vi "GOOP_VI_Item_OnPopupMenu.vi"(11 "Object":u64) -> ()   [LabVIEW 2020]
uses:
  <resource>/Framework/Providers/API/mxLvMenuItem.ctl
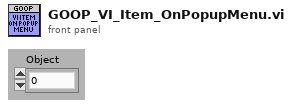
[diagram p1: front panel]
types:
  T1 = typedef "mxLvMenuItem.ctl" = cluster{"Menu Name":string, "Description":string, "Icon File Name":path, "Menu Tag":string, "Enabled":bool, "Checked":bool, "Separator":bool, "Batchable":bool, "Weight":i32, "Batch Mode (Ignored if Not Batchable)":enum32{"Show If All Items Support Command", "Show If Any Items Support Command"}, "Menu Location":enum32{"<None>", "Project", "Project / Build Specifications", "Tools", "Tools / Source Control", "Tools / Real-Time Module", "Help"}, "Exclude From Getting Started Window Menu":bool}
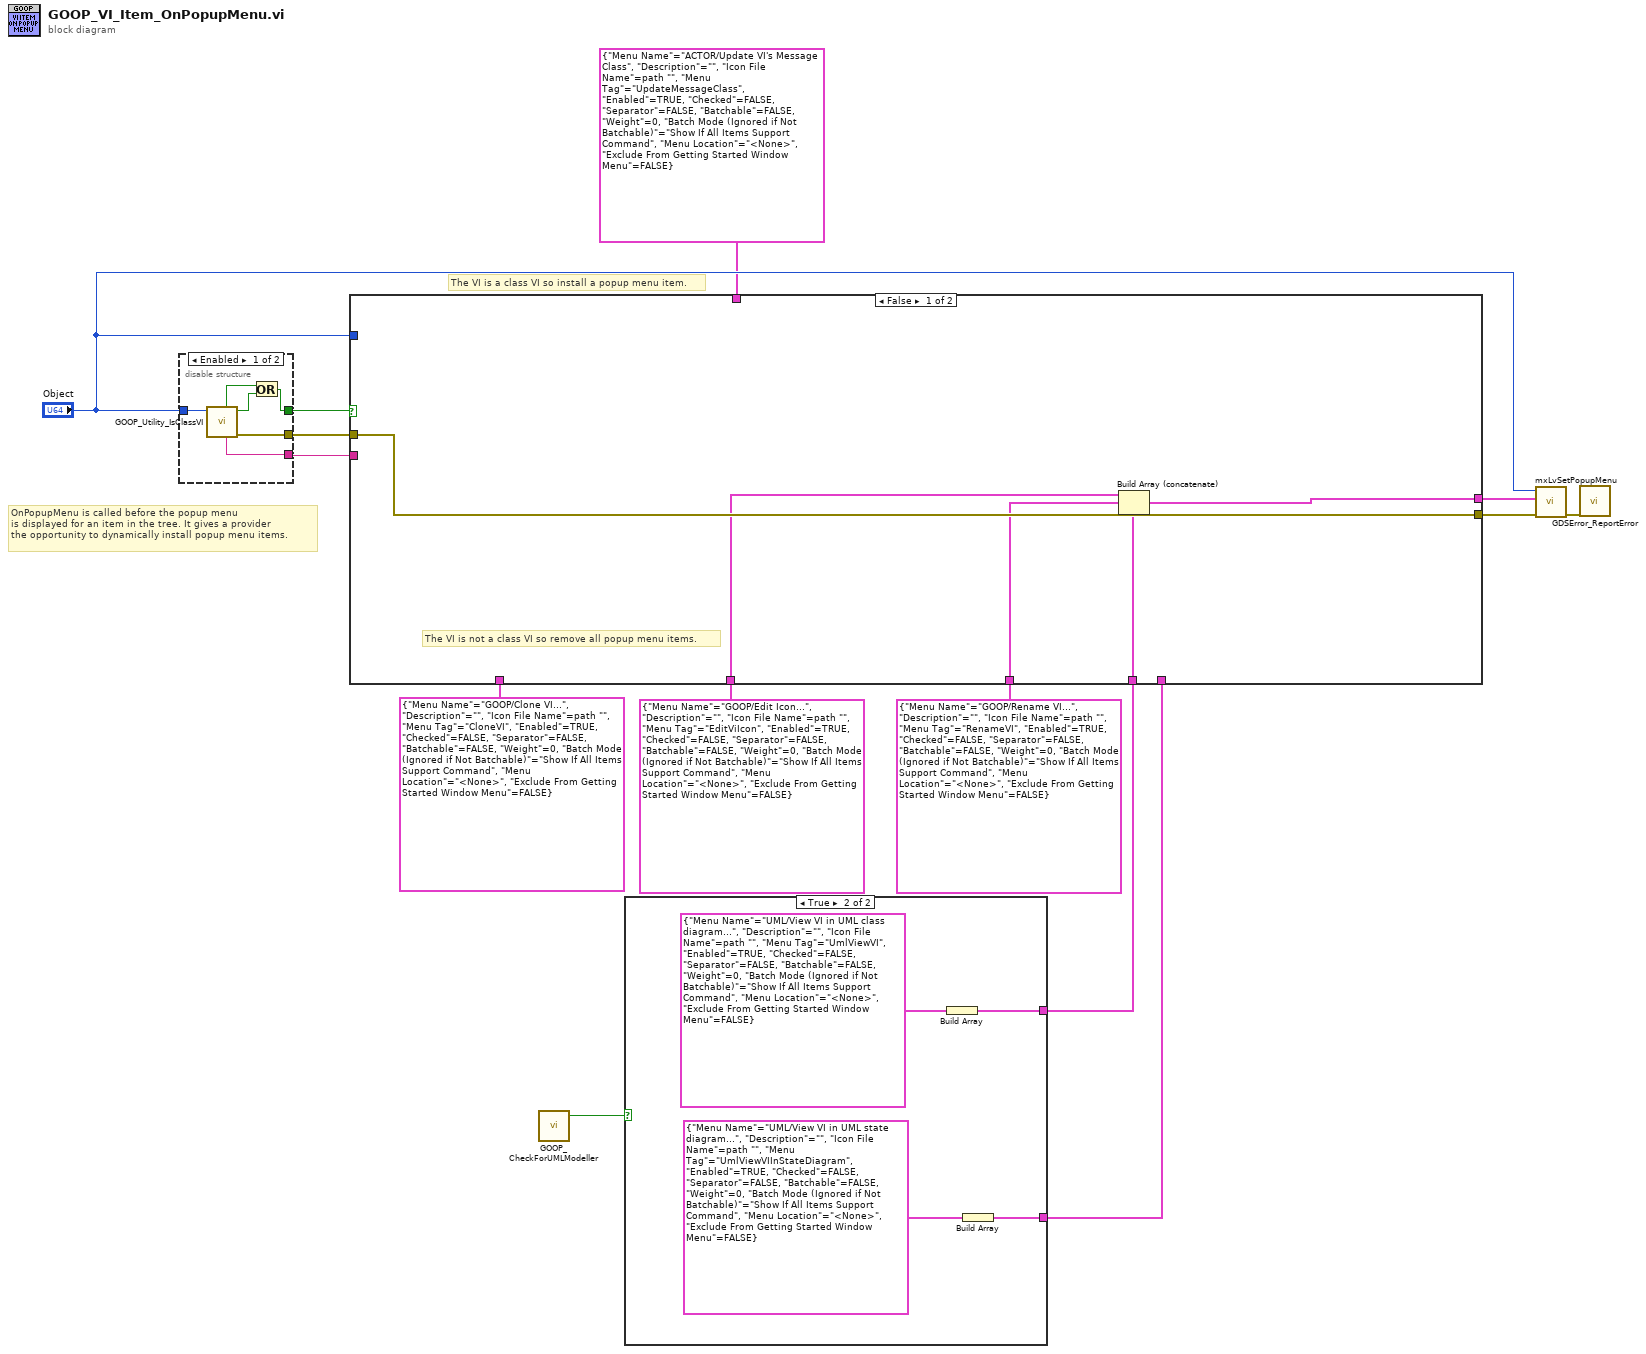
[diagram p0: block diagram]
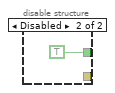
[diagram p3: hidden frame]
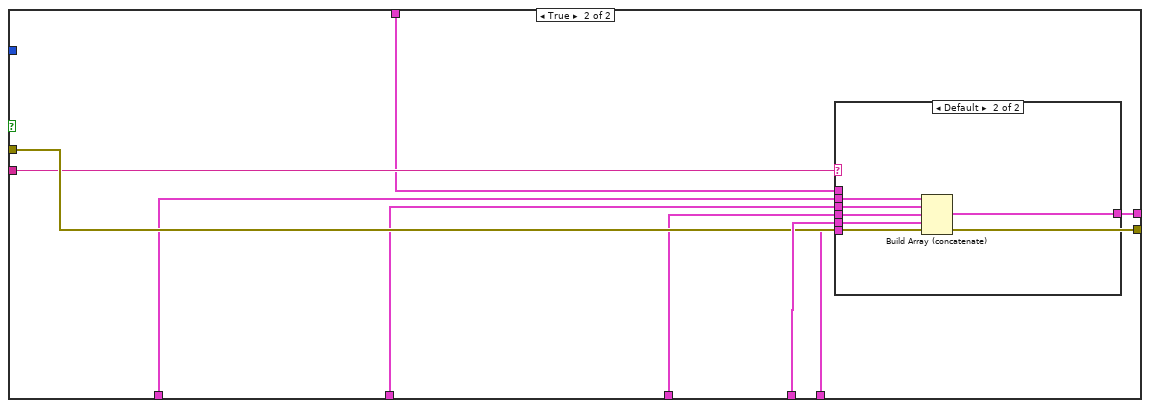
[diagram p4: hidden frame]
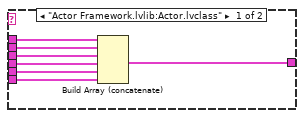
[diagram p5: hidden frame]
diagram:
  # "The VI is a class VI so install a popup menu item."
  # "OnPopupMenu is called before the popup menu\nis displayed for an item in the tree. It gives a provider\nthe opportunity to dynamically install popup menu items."
  n1 = disable-structure shown="Enabled" {
    disable-tunnel: "Object" -> [w20 _]
    disable-tunnel: [w19 _] -> w13
    disable-tunnel: [w15 TRUE ("Is Class VI?")] -> w11
    disable-tunnel: [w18 _] -> w7
    frame Enabled {
      n2 = call <resource>:"GOOP_Utility_IsClassVI.vi"("Object"=w20) -> ("error out"=w19:errorcluster, "Is Class VI?"=w16:bool, "RootClassQualified Class Name"=w18:string, "Is Interface?"=w17:bool)  [unwired: 5 in, 2 out]
      n3 = Or(x=w17, y=w16) -> (x .or. y?=w15:bool)
    }
    frame Disabled {
    }
  }
  n4 = call <resource>:"GOOP_CheckForUMLModeller.vi"() -> ("UML Modeller Exists"=w2:bool)  [unwired: 10 in, 1 out]
  n5 = case shown="True" w2 {
    tunnel: [_ w23] -> w4
    tunnel: [_ w22] -> w3
    frame False {
    }
    frame True {
      n6 = Build Array(T1 {"Menu Name"="UML/View VI in UML class diagram...", "Description"="", "Icon File Name"=path "", "Menu Tag"="UmlViewVI", "Enabled"=TRUE, "Checked"=FALSE, "Separator"=FALSE, "Batchable"=FALSE, "Weight"=0, "Batch Mode (Ignored if Not Batchable)"=enum."Show If All Items Support Command", "Menu Location"=enum."<None>", "Exclude From Getting Started Window Menu"=FALSE} ("Menu Item")) -> (w23:T1[])
      n7 = Build Array(T1 {"Menu Name"="UML/View VI in UML state diagram...", "Description"="", "Icon File Name"=path "", "Menu Tag"="UmlViewVIInStateDiagram", "Enabled"=TRUE, "Checked"=FALSE, "Separator"=FALSE, "Batchable"=FALSE, "Weight"=0, "Batch Mode (Ignored if Not Batchable)"=enum."Show If All Items Support Command", "Menu Location"=enum."<None>", "Exclude From Getting Started Window Menu"=FALSE} ("Menu Item")) -> (w22:T1[])
    }
  }
  n8 = case shown="False" w11 {
    tunnel: [w28 w37] -> w1
    tunnel: "Object" -> [_ _]
    tunnel: w13 -> [w30 w38]
    tunnel: w4 -> [w27 w39]
    tunnel: T1 {"Menu Name"="GOOP/Clone VI...", "Description"="", "Icon File Name"=path "", "Menu Tag"="CloneVI", "Enabled"=TRUE, "Checked"=FALSE, "Separator"=FALSE, "Batchable"=FALSE, "Weight"=0, "Batch Mode (Ignored if Not Batchable)"=enum."Show If All Items Support Command", "Menu Location"=enum."<None>", "Exclude From Getting Started Window Menu"=FALSE} ("Menu Item") -> [_ w36]
    tunnel: [w30 w38] -> w10
    tunnel: T1 {"Menu Name"="GOOP/Edit Icon...", "Description"="", "Icon File Name"=path "", "Menu Tag"="EditViIcon", "Enabled"=TRUE, "Checked"=FALSE, "Separator"=FALSE, "Batchable"=FALSE, "Weight"=0, "Batch Mode (Ignored if Not Batchable)"=enum."Show If All Items Support Command", "Menu Location"=enum."<None>", "Exclude From Getting Started Window Menu"=FALSE} ("Menu Item") -> [w29 w35]
    tunnel: w3 -> [_ w34]
    tunnel: w7 -> [_ w33]
    tunnel: T1 {"Menu Name"="ACTOR/Update VI's Message Class", "Description"="", "Icon File Name"=path "", "Menu Tag"="UpdateMessageClass", "Enabled"=TRUE, "Checked"=FALSE, "Separator"=FALSE, "Batchable"=FALSE, "Weight"=0, "Batch Mode (Ignored if Not Batchable)"=enum."Show If All Items Support Command", "Menu Location"=enum."<None>", "Exclude From Getting Started Window Menu"=FALSE} ("Menu Item") -> [_ w32]
    tunnel: T1 {"Menu Name"="GOOP/Rename VI...", "Description"="", "Icon File Name"=path "", "Menu Tag"="RenameVI", "Enabled"=TRUE, "Checked"=FALSE, "Separator"=FALSE, "Batchable"=FALSE, "Weight"=0, "Batch Mode (Ignored if Not Batchable)"=enum."Show If All Items Support Command", "Menu Location"=enum."<None>", "Exclude From Getting Started Window Menu"=FALSE} ("Menu Item") -> [w26 w31]
    frame False {
      # "The VI is not a class VI so remove all popup menu items."
      n9 = Build Array (concatenate)(w29, w26, w27) -> (w28:T1[])
    }
    frame True {
      n10 = case shown="Default" w33 {
        tunnel: w39 -> [w46 w52]
        tunnel: [w45 w51] -> w37
        tunnel: w36 -> [w44 w50]
        tunnel: w35 -> [w43 w49]
        tunnel: w34 -> [w42 w48]
        tunnel: w32 -> [w41 _]
        tunnel: w31 -> [w40 w47]
        frame "Actor Framework.lvlib:Actor.lvclass" {
          n11 = Build Array (concatenate)(w41, w44, w43, w40, w46, w42) -> (w45:T1[])
        }
        frame Default {
          n12 = Build Array (concatenate)(w50, w49, w47, w52, w48) -> (w51:T1[])
        }
      }
    }
  }
  n13 = call <resource>:"mxLvSetPopupMenu.vi"("error in"=w10, "Popup Menu Items"=w1, "Item"="Object") -> ("error out"=w9:errorcluster)  [unwired: 7 in, 1 out]
  n14 = call <resource>:"GDSError_ReportError.vi"("error in (no error)"=w9) -> ()  [unwired: 18 in, 1 out]
